vi "Browse for XNET Database.vi"(8 "error in (no error)":errorcluster) -> (0 "error out":errorcluster, 1 "Cancel Out":bool, 2 "Import Path out":path, 3 "XNET Settings":T1={"Database"="", "Cluster"="", "Port"="", "Baud rate [Bd]"=0, "Termination"=0, "CAN I/O Mode"=0, "FD Baud rate [Bd]"=500000, "Priority"=100, "Use Legacy"=FALSE, "FD ISO Mode"=0, "Default Max Counter Value"=0.0, "Default Protect Type"=enum."Arb ID + Bytes Checksum with Inversion", "Include All Channels"=FALSE} {"FD ISO Mode" items=["ISO", "Non ISO", "ISO Legacy"]; "CAN I/O Mode" items=["CAN 2.0", "CAN FD", "CAN FD+BRS"]; "Termination" items=["Off", "On"]})   [LabVIEW 2025, in "Protection and Counter Addon System Explorer.lvlib"]
uses:
  Protection and Counter Addon System Explorer.lvlib
  Addon Shared/Types/XNET Settings.ctl
  SubModules/Frame-Protection-Support/Source/Shared/Types/Protection Type.ctl
  <resource>/objmgr/xnet.rc
  Addon Shared/Protection and Counter Addon Shared.lvlib
  SubModules/Frame-Protection-Support/Source/Shared/Protection and Counter Support Shared.lvlib
panel:
  in  "Port":string="CAN1"
  in  "Path":path caption="Previous Personality Path (Optional)"
  in  "FD Baud rate [Bd]":u64=500000
  out "CAN I/O Mode":u32(ring) items=["CAN 2.0", "CAN FD", "CAN FD+BRS"]
  in  "Baud rate [Bd]":u64=500000
  in  "Select CAN Cluster":u16(ring)
  in  "Cancel":bool
  in  "Select":bool
  in  "XNET Database":refnum<k21>
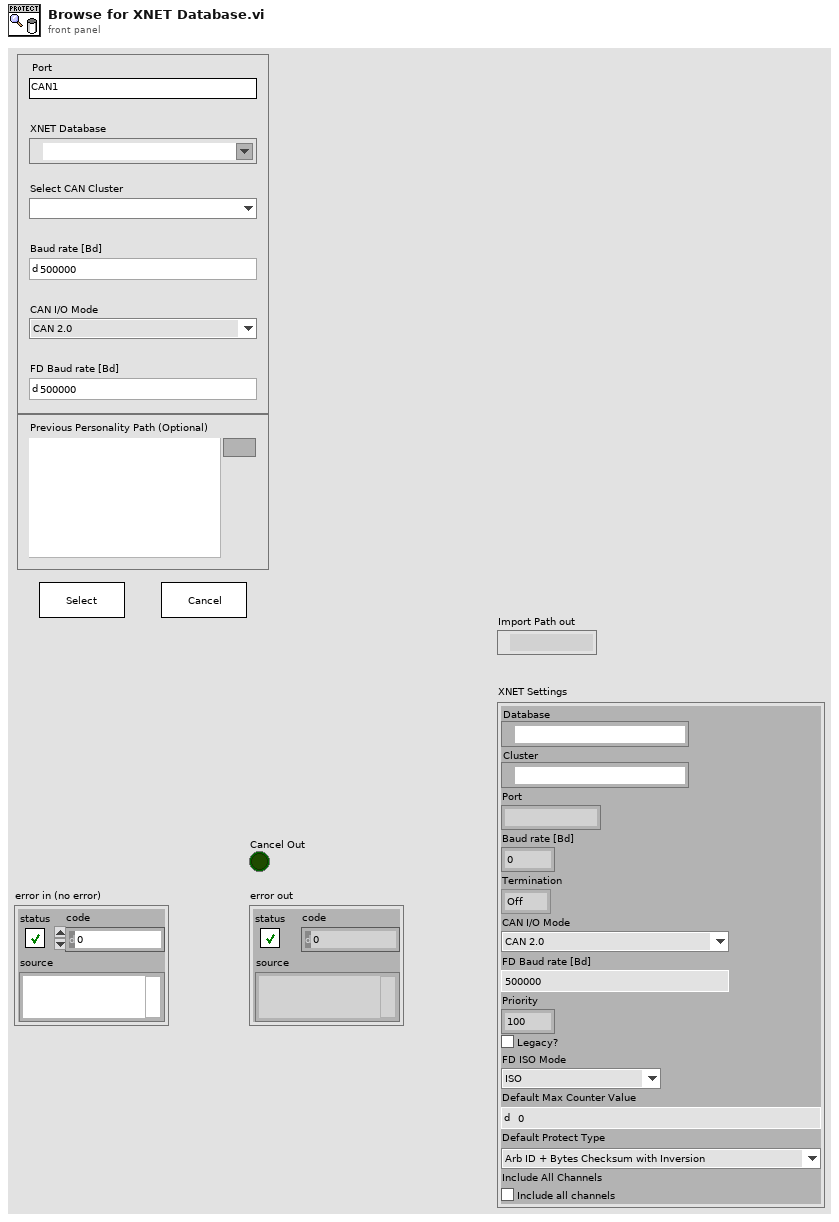
[diagram p1: front panel]
types:
  T1 = typedef "Protection and Counter Addon Shared.lvlib/XNET Settings.ctl" = cluster{"Database":refnum<k21>, "Cluster":refnum<k21>, "Port":string, "Baud rate [Bd]":u64, "Termination":u32, "CAN I/O Mode":u32, "FD Baud rate [Bd]":u64, "Priority":i32, "Use Legacy":bool, "FD ISO Mode":u32, "Default Max Counter Value":dbl, "Default Protect Type":T2, "Include All Channels":bool}
  T2 = typedef "Protection and Counter Support Shared.lvlib/Protection Type.ctl" = enum16{"Arb ID + Bytes Checksum with Inversion", "Arb ID + Bytes CRC with Inversion", "Reversed Raw Signal Checksum with Inversion", "Concatenated Two's Compliment"}
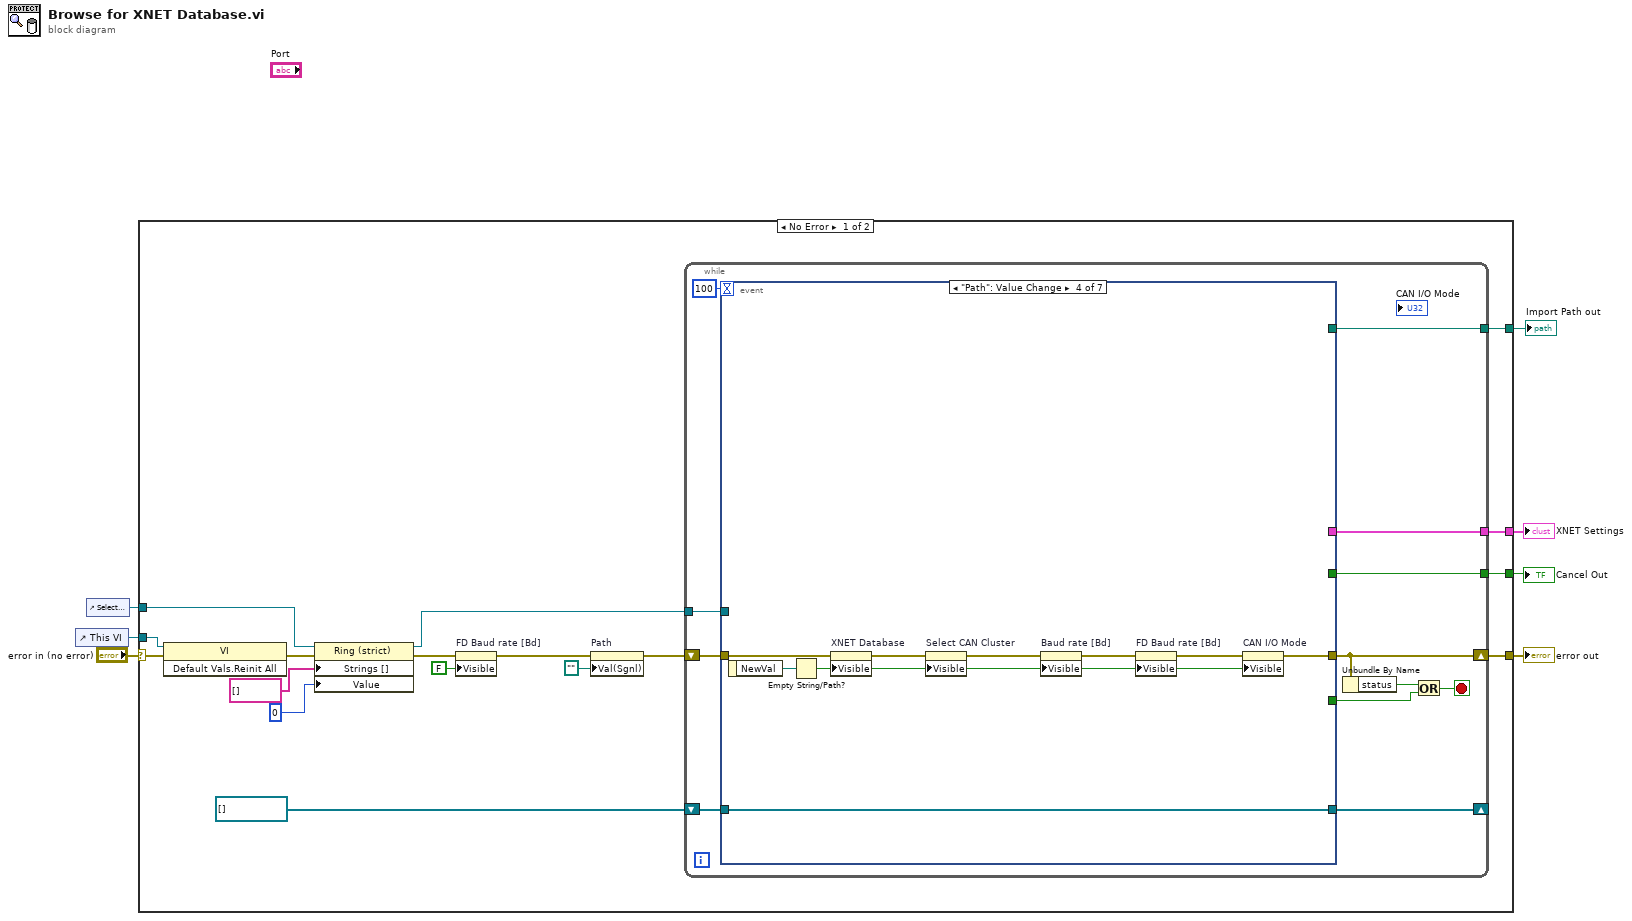
[diagram p0: block diagram]
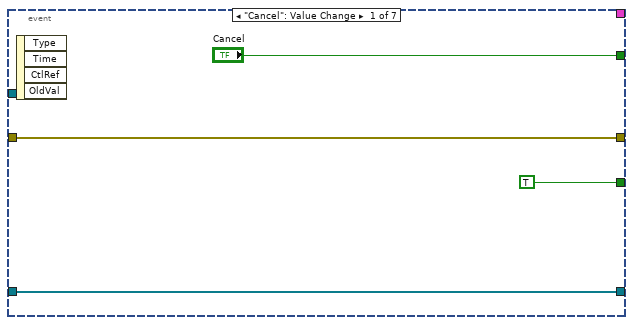
[diagram p2: hidden frame]
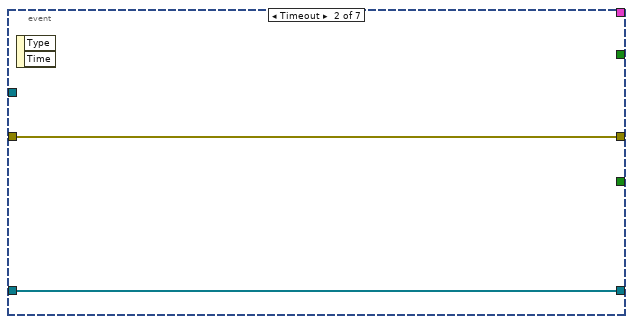
[diagram p3: hidden frame]
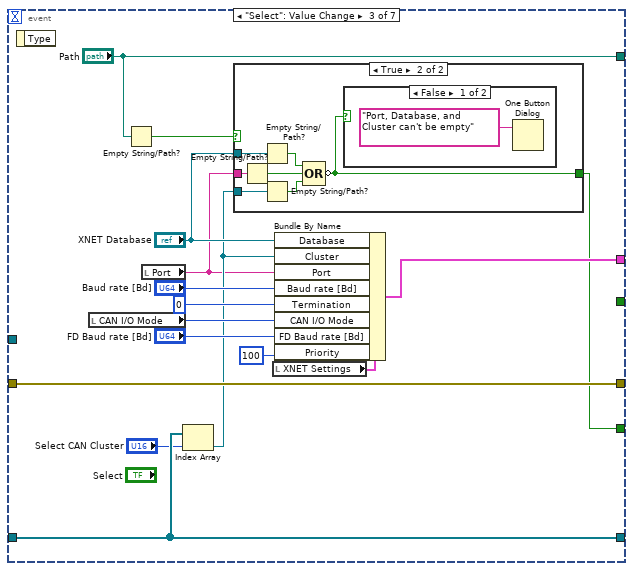
[diagram p4: hidden frame]
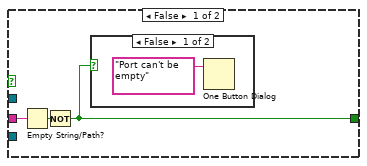
[diagram p5: hidden frame]
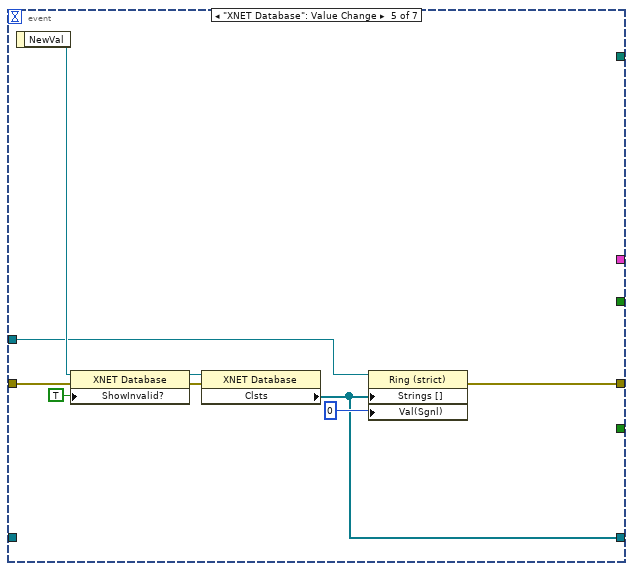
[diagram p8: hidden frame]
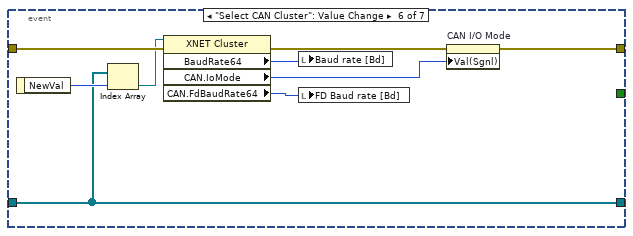
[diagram p9: hidden frame]
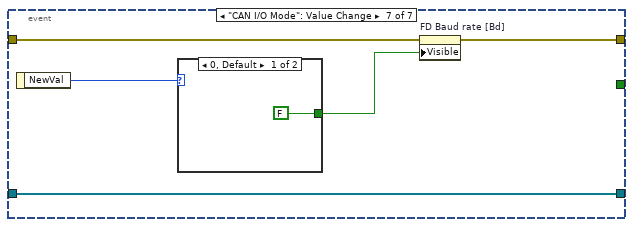
[diagram p10: hidden frame]
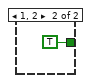
[diagram p11: hidden frame]
diagram:
  n1 = control-ref of="This VI"() -> (w4:refnum<vi>)
  n2 = control-ref of="Select CAN Cluster"() -> (w2:refnum<vi>)
  n3 = case shown="No Error" "error in (no error)" {
    selector: "error in (no error)" -> [w23 w105]
    tunnel: [w21 w105] -> w6
    tunnel: [w24 _] -> w5
    tunnel: w4 -> [w22 _]
    tunnel: [w19 _] -> w3
    tunnel: w2 -> [w18 _]
    tunnel: [w11 _] -> w1
    frame No Error {
      n4 = invoke class="VI" method="Default Vals.Reinit All"(reference=w22, error in=w23) -> (error out=w17:errorcluster)  [unwired: 1 in, 2 out]
      n5 = property on="Property Node" class="Ring (strict)"(reference=w18, error in=w17, "Strings []"=string[] [], "Value"=u16 0) -> (reference out=w16:refnum<vi>, error out=w13:errorcluster)
      n6 = property on="FD Baud rate [Bd]" class="DigNum (strict)"(error in=w13, "Visible"=FALSE) -> (error out=w10:errorcluster)  [unwired: 1 in, 1 out]
      n7 = property on="Path" class="Path"(error in=w10, "Val(Sgnl)"=path "") -> (error out=w9:errorcluster)  [unwired: 1 in, 1 out]
      n8 = while {
        tunnel: [w36] -> w24
        shift-right: [w34] -> _
        shift-left: refnum<k21>[] [] ("Clsts") -> [w33]
        shift-right: [w30] -> w21
        shift-left: w9 -> [w35]
        tunnel: [w32] -> w19
        tunnel: w16 -> [w26]
        tunnel: [w25] -> w11
        stop <- w27 stop-if-true
        n9 = event shown="[3] \"Path\": Value Change" {
          selector: _ -> [_ _ _ _ _ _ _]
          dyn-events: _ -> [_ _ _ _ _ _ _]
          timeout: 100 -> [_ _ _ _ _ _ _]
          tunnel: ["Cancel" _ _ _ _ _ _] -> w36
          tunnel: w35 -> [w38 w42 w53 w76 w85 w96 w102]
          tunnel: [w39 w41 w57 w79 w82 w93 w100] -> w34
          tunnel: w33 -> [w39 w41 w57 w79 _ w93 w100]
          tunnel: [w38 w42 w53 w72 w80 w91 w101] -> w30
          tunnel: [_ _ w55 _ _ _ _] -> w32
          tunnel: [TRUE _ w43 _ _ _ _] -> w28
          tunnel: w26 -> [_ _ _ _ w81 _ _]
          tunnel: [_ _ "Path" _ _ _ _] -> w25
          event "Cancel": Value Change {
            n10 = event-data() -> ()  [unwired: 1 in, 4 out]
          }
          event Timeout {
            n11 = event-data() -> ()  [unwired: 1 in, 2 out]
          }
          event "Select": Value Change {
            n12 = event-data() -> ()  [unwired: 1 in, 1 out]
            n13 = local read "CAN I/O Mode"() -> (w51:u32)
            n14 = Empty String/Path?(string/path="Path") -> (empty?=w44:bool)
            n15 = local read "Port"() -> (w48:string)
            n16 = Index Array(array=w57, index="Select CAN Cluster") -> (element=w49:refnum<k21>)
            n17 = case shown="True" w44 {
              tunnel: "XNET Database" -> [_ w69]
              tunnel: w49 -> [_ w68]
              tunnel: w48 -> [w61 w67]
              tunnel: [w59 w63] -> w43
              frame False {
                n18 = Empty String/Path?(string/path=w61) -> (empty?=w60:bool)
                n19 = Not(x=w60) -> (.not. x?=w59:bool)
                n20 = case shown="False" w59 {
                  frame False {
                    n21 = One Button Dialog(message="Port can't be empty") -> ()  [unwired: 1 in, 1 out]
                  }
                  frame True {
                  }
                }
              }
              frame True {
                n22 = Empty String/Path?(string/path=w67) -> (empty?=w65:bool)
                n23 = Empty String/Path?(string/path=w69) -> (empty?=w66:bool)
                n24 = Empty String/Path?(string/path=w68) -> (empty?=w64:bool)
                n25 = Compound Arithmetic op=OR(w66, w65, w64) -> (invert w63:bool)
                n26 = case shown="False" w63 {
                  frame False {
                    n27 = One Button Dialog(message="Port, Database, and Cluster can't be empty") -> ()  [unwired: 1 in, 1 out]
                  }
                  frame True {
                  }
                }
              }
            }
            n28 = local read "XNET Settings"() -> (w46:T1)
            n29 = Bundle By Name(cluster=w46, "Database"="XNET Database", "Cluster"=w49, "Port"=w48, "Baud rate [Bd]"="Baud rate [Bd]", "Termination"=u32 0, "CAN I/O Mode"=w51, "FD Baud rate [Bd]"="FD Baud rate [Bd]", "Priority"=100) -> (w55:T1)
          }
          event "Path": Value Change {
            n30 = event-data() -> ("NewVal"=w78:path)  [unwired: 1 in]
            n31 = Empty String/Path?(string/path=w78) -> (empty?=w71:bool)
            n32 = property on="XNET Database" class="XNET (strict)"(error in=w76, "Visible"=w71) -> (error out=w77:errorcluster)  [unwired: 1 in, 1 out]
            n33 = property on="Select CAN Cluster" class="Ring (strict)"(error in=w77, "Visible"=w71) -> (error out=w74:errorcluster)  [unwired: 1 in, 1 out]
            n34 = property on="Baud rate [Bd]" class="DigNum (strict)"(error in=w74, "Visible"=w71) -> (error out=w75:errorcluster)  [unwired: 1 in, 1 out]
            n35 = property on="FD Baud rate [Bd]" class="DigNum (strict)"(error in=w75, "Visible"=w71) -> (error out=w73:errorcluster)  [unwired: 1 in, 1 out]
            n36 = property on="CAN I/O Mode" class="Ring (strict)"(error in=w73, "Visible"=w71) -> (error out=w72:errorcluster)  [unwired: 1 in, 1 out]
          }
          event "XNET Database": Value Change {
            n37 = event-data() -> ("NewVal"=w84:refnum<k21>)  [unwired: 1 in]
            n38 = property class="XNET Database"(reference=w84, error in=w85, "ShowInvalid?"=TRUE ("Show Invalid From Open?")) -> (reference out=w88:refnum<k21>, error out=w87:errorcluster)
            n39 = property class="XNET Database"(reference=w88, error in=w87) -> ("Clsts"=w82:refnum<k21>[])  [unwired: 2 out]
            n40 = property on="Property Node" class="Ring (strict)"(reference=w81, "Strings []"=w82, "Val(Sgnl)"=u16 0 ("Value (Signaling)")) -> (error out=w80:errorcluster)  [unwired: 1 in, 1 out]
          }
          event "Select CAN Cluster": Value Change {
            n41 = event-data() -> ("NewVal"=w95:u16)  [unwired: 1 in]
            n42 = Index Array(array=w93, index=w95) -> (element=w94:refnum<k21>)
            n43 = property class="XNET Cluster"(reference=w94, error in=w96) -> (error out=w90:errorcluster, "BaudRate64"=w97:u64, "CAN.IoMode"=w89:u32, "CAN.FdBaudRate64"=w92:u64)  [unwired: 1 out]
            n44 = local write "Baud rate [Bd]"(w97) -> ()
            n45 = local write "FD Baud rate [Bd]"(w92) -> ()
            n46 = property on="CAN I/O Mode" class="Ring (strict)"(error in=w90, "Val(Sgnl)"=w89) -> (error out=w91:errorcluster)  [unwired: 1 in, 1 out]
          }
          event "CAN I/O Mode": Value Change {
            n47 = event-data() -> ("NewVal"=w98:u32)  [unwired: 1 in]
            n48 = case shown="0, Default" w98 {
              tunnel: [FALSE TRUE] -> w99
              frame 0, Default {
              }
              frame 1, 2 {
              }
            }
            n49 = property on="FD Baud rate [Bd]" class="DigNum (strict)"(error in=w102, "Visible"=w99) -> (error out=w101:errorcluster)  [unwired: 1 in, 1 out]
          }
        }
        n50 = Unbundle By Name(w30) -> ("status"=w29:bool)
        n51 = Or(x=w29, y=w28) -> (x .or. y?=w27:bool)
      }
    }
    frame Error {
    }
  }
  "error out" <- w6
  "Cancel Out" <- w5
  "XNET Settings" <- w3
  "Import Path out" <- w1
